vi "Parse Default Request.vi"(8 "error in (no error)":errorcluster caption="에러 입력(에러 없음)", 10 "JSON string":string, 11 "Instrument Manager 입력":refnum<class "Instrument Manager.lvclass">) -> (0 "error out":errorcluster caption="에러 출력", 2 "Default Request":T1, 3 "Instrument Manager 출력":refnum<class "Instrument Manager.lvclass">)   [LabVIEW 2023, in "Instrument Manager.lvclass"]
uses:
  Instrument Manager.lvclass
  Default Request.ctl
  Instrument Manager.lvclass/Instrument Manager.ctl
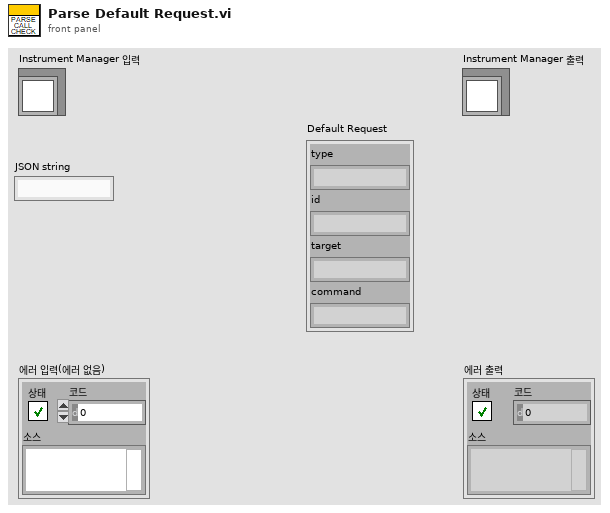
[diagram p1: front panel]
types:
  T1 = typedef "Instrument Manager.lvclass/Default Request.ctl" = cluster{"type":string, "id":string, "target":string, "command":string}
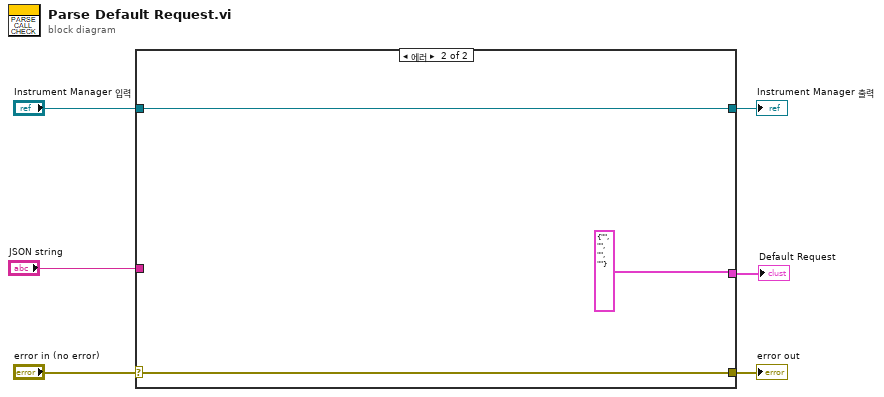
[diagram p0: block diagram]
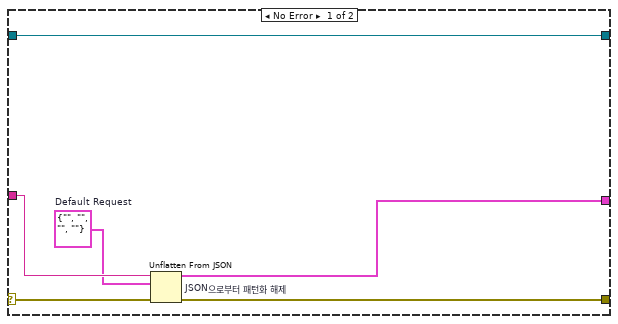
[diagram p2: hidden frame]
diagram:
  n1 = case shown="에러" "error in (no error)" {
    selector: "error in (no error)" -> [w11 w15]
    tunnel: [w7 w15] -> w5
    tunnel: [w12 w14] -> w3
    tunnel: "Instrument Manager 입력" -> [w12 w14]
    tunnel: "JSON string" -> [w10 _]
    tunnel: [w8 T1 {"type"="", "id"="", "target"="", "command"=""} ("Default Request")] -> w1
    frame No Error {
      w9 = T1 {"type"="", "id"="", "target"="", "command"=""}  # Default Request
      n2 = Unflatten From JSON "JSON으로부터 패턴화 해제"(JSON string=w10, type and defaults=w9, error in (no error)=w11) -> (value=w8:T1, error out=w7:errorcluster)  [unwired: 4 in]
    }
    frame Error {
    }
  }
  "error out" <- w5
  "Instrument Manager 출력" <- w3
  "Default Request" <- w1
